vi "Create.vi"(7 "Direction":T1, 8 "error in (no error)":errorcluster, 9 "Custom Config Data":u8[](array[numeric]), 10 "Name":string, 11 "CIFFIFO in":refnum<class "CIF_CIPC_Fifo_DAQ.lvclass">) -> (0 "error out":errorcluster, 3 "CIFFIFO out":refnum<class "CIF_CIPC_Fifo_DAQ.lvclass">)   [LabVIEW 2021, in "CIF_CIPC_Fifo_DAQ.lvclass"]
uses:
  CIF_CIPC_Fifo_DAQ.lvclass
  <vilib>/CIF Foundation/CIF Channels Core/ChannelCommon/typedef/Direction.ctl
  C:/Program Files/National Instruments/LabVIEW 2021/vi.lib/CIF Foundation/CIF Channels Core/CIFChannels/CIFChannels.lvclass
  D:/dev/Packages/CIF_Channels_CIPC/src/CIPC_Channels/CIF_CIPC_Chan/CIF_CIPC_Chn.lvclass
  <vilib>/CIF Foundation/CIF Utilities/Statistics/I64/Stats_I64_CIF_U.lvclass/Stats_I64_CIF_U.ctl
  <vilib>/CIF Foundation/CIF Channels Core/ChannelCommon/typedef/Channel State.ctl
  <vilib>/CIF Foundation/CIF Channels Core/ChannelCommon/typedef/Disconnect Behavior.ctl
  <vilib>/CIF Foundation/CIF Channels Core/CIFChannels/CIFChannels.lvclass/CIFChannels.ctl
  <vilib>/CIF Foundation/CIF Channels Core/ChannelCommon/typedef/Channel Pattern.ctl
  CIF_CIPC_Chan/Typedef/Buffer Configuration Data.ctl
  <vilib>/CIF Foundation/CIF CIPC/TypeDefs/Backpressure References.ctl
  <vilib>/CIF Foundation/CIF CIPC/TypeDefs/Backpressure Names.ctl
  CIF_CIPC_Chan/CIF_CIPC_Chn.lvclass/CIF_CIPC_Chn.ctl
  35849dc3-58aa-4d75-b906-fe3df34869a7.vi
  <vilib>/CIF Foundation/CIF Channels Core/CIFChannels/Accessors/Write Pattern.vi
  CIF_CIPC_Chan/Accessors/Write Buffer Configuration.vi
  CIF_CIPC_Chan/Accessors/Write CIPC Channel.vi
  9be4d617-3037-4515-bcea-2a1e3727d04e.vi
  <vilib>/CIF Foundation/CIF Channels Core/CIFChannels/Accessors/Write Channel State.vi
  <vilib>/CIF Foundation/CIF Channels Core/CIFChannels/Accessors/Write Subscriber Count.vi
  <vilib>/CIF Foundation/CIF Channels Core/CIFChannels/Accessors/Write Channel Benchmark.vi
  <vilib>/CIF Foundation/CIF Channels Core/CIFChannels/Accessors/Write Flatten Benchmark.vi
  35849dc3-58aa-4d75-b906-fe3df34869a7.vi/bd07d5d9-1209-45ad-b636-9e9ab86132fb.vi
  <vilib>/CIF Foundation/CIF CIPC/SubVIs/Check Error.vi
  <vilib>/CIF Foundation/CIF CIPC/SubVIs/Add CIPC Error.vi
  <vilib>/CIF Foundation/CIF CIPC/SubVIs/Get dll Path.vi
  9be4d617-3037-4515-bcea-2a1e3727d04e.vi/49b3dd2d-4579-4089-b72e-3f0875c862f2.vi
  9be4d617-3037-4515-bcea-2a1e3727d04e.vi/1e2c93d0-55b0-4d6c-a9da-21395a664279.vi
  9be4d617-3037-4515-bcea-2a1e3727d04e.vi/7bb13226-97f3-4dcb-9346-06ec631a2876.vi
  9be4d617-3037-4515-bcea-2a1e3727d04e.vi/49b3dd2d-4579-4089-b72e-3f0875c862f2.vi/bd07d5d9-1209-45ad-b636-9e9ab86132fb.vi
  9be4d617-3037-4515-bcea-2a1e3727d04e.vi/1e2c93d0-55b0-4d6c-a9da-21395a664279.vi/49b3dd2d-4579-4089-b72e-3f0875c862f2.vi
  <vilib>/CIF Foundation/CIF CIPC/SubVIs/Notify Of New Write.vi
  <vilib>/CIF Foundation/CIF CIPC/SubVIs/Get Element Write Position.vi
  <vilib>/CIF Foundation/CIF CIPC/SubVIs/Get Element Description Variant.vi
  <vilib>/Utility/error.llb/Trim Whitespace.vi
  <vilib>/string/Create NI GUID.vi
  <vilib>/CIF Foundation/CIF CIPC/SubVIs/Check Error Core.vi
  <vilib>/CIF Foundation/CIF CIPC/SubVIs/Add CIPC Error Core.vi
  <vilib>/CIF Foundation/CIF CIPC/SubVIs/Get Backpressure Name.vi
  <vilib>/CIF Foundation/CIF CIPC/SubVIs/Get Element Info Variant.vi
  <vilib>/CIF Foundation/CIF Utilities/Statistics/I64/Stats_I64_CIF_U.lvclass
  <vilib>/CIF Foundation/CIF Channels Core/CIFChannels/CIFChannels.lvclass
  <vilib>/CIF Foundation/CIF Channels Core/ChannelCommon/ChannelCommon.lvlib
  <vilib>/CIF Foundation/CIF CIPC/CIF_NI_CIPC.lvlib
  CIF_CIPC_Chan/CIF_CIPC_Chn.lvclass
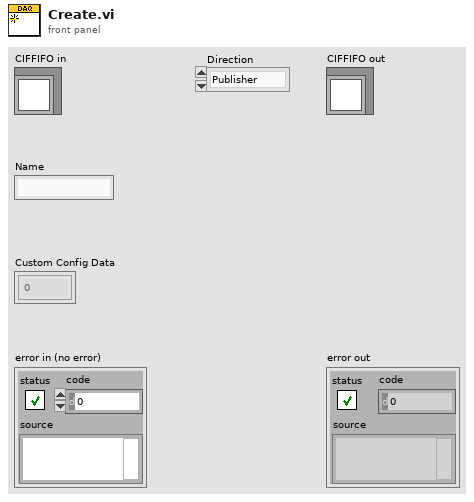
[diagram p1: front panel]
types:
  T1 = typedef "ChannelCommon.lvlib/Direction.ctl" = enum8{"Publisher", "Subscriber"}
  T2 = typedef "ChannelCommon.lvlib/Channel State.ctl" = enum8{"Creating", "Disconnected", "Connecting", "Connected", "Destroyed"}
  T3 = typedef "ChannelCommon.lvlib/Disconnect Behavior.ctl" = enum8{"Default value", "Last value", "Error with default"}
  T4 = typedef "ChannelCommon.lvlib/Channel Pattern.ctl" = enum8{"Unknown", "Tag", "FIFO", "MultiFIFO", "BackpressureFIFO"}
  T5 = typedef "CIF_CIPC_Chn.lvclass/Buffer Configuration Data.ctl" = cluster{"Total Size":u32, "Read Size":u32, "Read Offset":u32, "CIPC BP References":T6, "CIPC Backpressure Names":T7, "Override CIPC Name":string, "Encoder Data":string}
  T6 = typedef "CIF_NI_CIPC.lvlib/Backpressure References.ctl" = cluster{"CIPC Reference":u64, "CIPC BP Reference":u64}
  T7 = typedef "CIF_NI_CIPC.lvlib/Backpressure Names.ctl" = cluster{"CIPC Name":string, "CIPC BP Name":string}
  T8 = typedef "CIF_NI_CIPC.lvlib/Encoder Info.ctl" = cluster{"Name":string, "Version":i32, "Data":string}
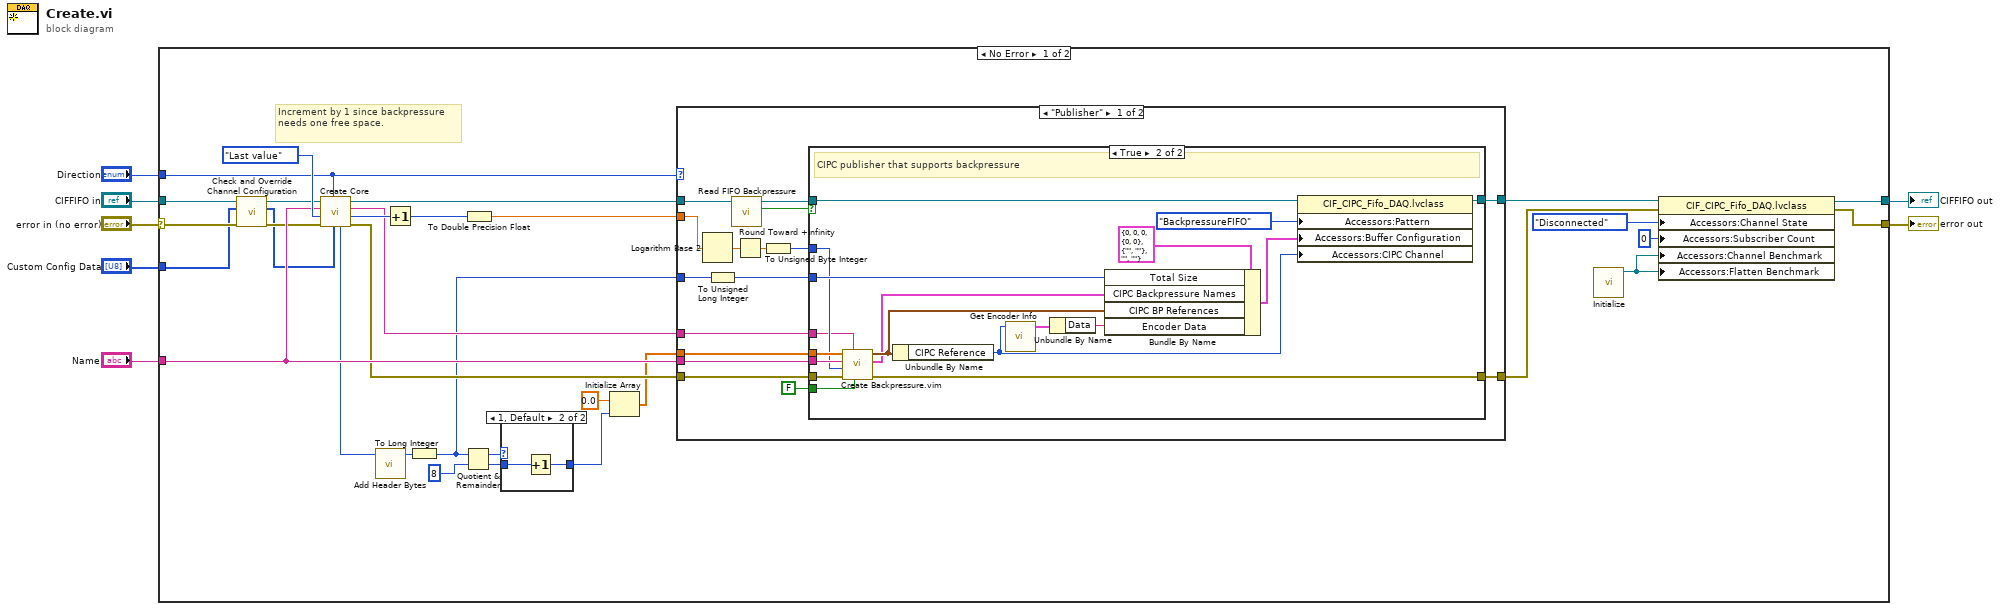
[diagram p0: block diagram]
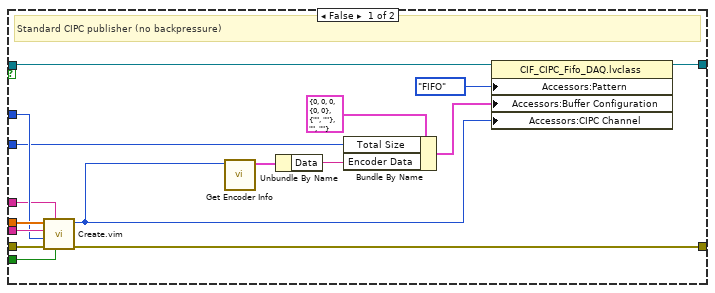
[diagram p3: hidden frame]
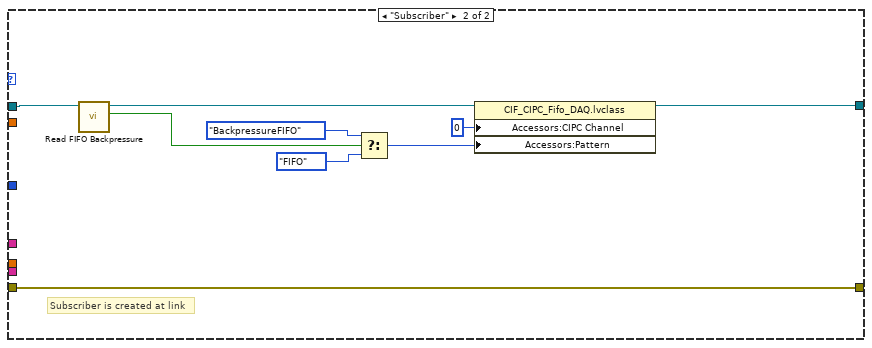
[diagram p4: hidden frame]
diagram:
  n1 = case shown="No Error" "error in (no error)" {
    selector: "error in (no error)" -> [w28 w102]
    tunnel: [w37 w102] -> w6
    tunnel: [w33 w101] -> w1
    tunnel: "CIFFIFO in" -> [w29 w101]
    tunnel: "Name" -> [w36 _]
    tunnel: "Direction" -> [w32 _]
    tunnel: "Custom Config Data" -> [w25 _]
    frame No Error {
      # "Increment by 1 since backpressure needs one free space."
      n2 = call-dynamic "Check and Override Channel Configuration.vi"("error in (no error)"=w28, "Custom Config Data in"=w25, "CIFFIFO in"=w29) -> ("error out"=w26:errorcluster, "Custom Config Data out"=w24:u8[], "CIFFIFO out"=w27:refnum<class "CIF_CIPC_Fifo_DAQ.lvclass">)  [unwired: 6 in]
      n3 = call <vilib>:"Create Core.vi"("Custom Config Data"=w24, "Direction"=w32, "error in (no error)"=w26, "Disconnect Behavior"=Disconnect_Behavior."Last value", "Name"=w36, "CIFChannels in"=w27) -> ("error out"=w35:errorcluster, "Messages"=w19:u64, "Channel Type"=w17:string, "CIFChannels out"=w21:refnum<class "CIF_CIPC_Fifo_DAQ.lvclass">, "Bytes/Msg"=w16:u64)  [unwired: 1 in]
      n4 = call <vilib>:"Add Header Bytes.vi"("Bytes/Msg"=w16) -> ("Bytes/Msg with header"=w20:u64)  [unwired: 3 in]
      n5 = Increment(x=w19) -> (x+1=w18:u64)
      n6 = To Long Integer(number=w20) -> (32bit integer=w15:i32)
      n7 = Quotient & Remainder(x=w15, y=8) -> (x-y*floor(x/y)=w13:i32, floor(x/y)=w12:i32)
      n8 = To Double Precision Float(number=w18) -> (double precision float=w22:dbl)
      n9 = case shown="1, Default" w13 {
        tunnel: w12 -> [w39 w41]
        tunnel: [w39 w40] -> w11
        frame 0 {
        }
        frame 1, Default {
          n10 = Increment(x=w41) -> (x+1=w40:i32)
        }
      }
      n11 = Initialize Array(0.0 ("Numeric"), w11) -> (w23:dbl[])
      n12 = case shown="\"Publisher\"" w32 {
        tunnel: w36 -> [w54 _]
        tunnel: w35 -> [w56 w100]
        tunnel: [w57 w100] -> w34
        tunnel: w22 -> [w51 _]
        tunnel: w23 -> [w53 _]
        tunnel: w21 -> [w48 w94]
        tunnel: w15 -> [w45 _]
        tunnel: [w43 w99] -> w10
        tunnel: w17 -> [w42 _]
        frame "Publisher" {
          n13 = Logarithm Base 2(1:w51) -> (0:w52:dbl)
          n14 = To Unsigned Long Integer(number=w45) -> (unsigned 32bit integer=w44:u32)
          n15 = call <vilib>:"Read FIFO Backpressure.vi"("CIFChannels in"=w48) -> ("Backpressure"=w46:bool, "CIFChannels out"=w47:refnum<class "CIF_CIPC_Fifo_DAQ.lvclass">)  [unwired: 8 in, 1 out]
          n16 = Round Toward +Infinity(x=w52) -> (ceil(x): smallest int >= x=w50:dbl)
          n17 = To Unsigned Byte Integer(number=w50) -> (unsigned 8bit integer=w49:u8)
          n18 = case shown="True" w46 {
            tunnel: [w73 w80] -> w57
            tunnel: w56 -> [w72 w81]
            tunnel: FALSE ("Prepend Array Size") -> [w71 w84]
            tunnel: w54 -> [w70 w83]
            tunnel: w53 -> [w69 w85]
            tunnel: w49 -> [w68 w82]
            tunnel: w47 -> [w67 w91]
            tunnel: w44 -> [w65 w89]
            tunnel: [w61 w86] -> w43
            tunnel: w42 -> [w60 w77]
            frame False {
              # "Standard CIPC publisher (no backpressure)"
              n19 = call "Create.vim"("Prepend Array Size"=w71, "Description"=w60, "error in (no error)"=w72, "Buffer Size N (2^N)"=w68, "Name in"=w70, "Data Type"=w69) -> ("error out"=w73:errorcluster, "CIPC Reference"=w62:u64)  [unwired: 2 in, 2 out]
              n20 = call <vilib>:"Get Encoder Info.vi"("CIPC Reference"=w62) -> ("Encoder Info"=w64:T8)  [unwired: 9 in, 1 out]
              n21 = Unbundle By Name(w64) -> ("Data"=w63:string)
              n22 = Bundle By Name(cluster=T5 {"Total Size"=0, "Read Size"=0, "Read Offset"=0, "CIPC BP References"={"CIPC Reference"=0, "CIPC BP Reference"=0}, "CIPC Backpressure Names"={"CIPC Name"="", "CIPC BP Name"=""}, "Override CIPC Name"="", "Encoder Data"=""} ("Buffer Configuration"), "Total Size"=w65, "Encoder Data"=w63) -> (w59:T5)
              n23 = property class="CIF_CIPC_Fifo_DAQ.lvclass"(reference=w67, "Accessors:Pattern"=Channel_Pattern."FIFO" ("Pattern"), "Accessors:Buffer Configuration"=w59, "Accessors:CIPC Channel"=w62) -> (reference out=w61:refnum<class "CIF_CIPC_Fifo_DAQ.lvclass">)  [unwired: 1 in, 1 out]
            }
            frame True {
              # "CIPC publisher that supports backpressure"
              n24 = call "Create Backpressure.vim"("Prepend Array Size"=w84, "Description"=w77, "error in (no error)"=w81, "Buffer Size N (2^N)"=w82, "Name in"=w83, "Data Type"=w85) -> ("error out"=w80:errorcluster, "CIPC Backpressure Names"=w74:T7, "CIPC BP References"=w78:T6)  [unwired: 2 in, 1 out]
              n25 = Unbundle By Name(w78) -> ("CIPC Reference"=w79:u64)
              n26 = call <vilib>:"Get Encoder Info.vi"("CIPC Reference"=w79) -> ("Encoder Info"=w88:T8)  [unwired: 9 in, 1 out]
              n27 = Unbundle By Name(w88) -> ("Data"=w87:string)
              n28 = Bundle By Name(cluster=T5 {"Total Size"=0, "Read Size"=0, "Read Offset"=0, "CIPC BP References"={"CIPC Reference"=0, "CIPC BP Reference"=0}, "CIPC Backpressure Names"={"CIPC Name"="", "CIPC BP Name"=""}, "Override CIPC Name"="", "Encoder Data"=""} ("Buffer Configuration"), "Total Size"=w89, "CIPC Backpressure Names"=w74, "CIPC BP References"=w78, "Encoder Data"=w87) -> (w76:T5)
              n29 = property class="CIF_CIPC_Fifo_DAQ.lvclass"(reference=w91, "Accessors:Pattern"=Channel_Pattern."BackpressureFIFO" ("Pattern"), "Accessors:Buffer Configuration"=w76, "Accessors:CIPC Channel"=w79) -> (reference out=w86:refnum<class "CIF_CIPC_Fifo_DAQ.lvclass">)  [unwired: 1 in, 1 out]
            }
          }
        }
        frame "Subscriber" {
          # "Subscriber is created at link"
          n30 = call <vilib>:"Read FIFO Backpressure.vi"("CIFChannels in"=w94) -> ("Backpressure"=w95:bool, "CIFChannels out"=w93:refnum<class "CIF_CIPC_Fifo_DAQ.lvclass">)  [unwired: 8 in, 1 out]
          n31 = Select(t=Channel_Pattern."BackpressureFIFO" ("Pattern"), s=w95, f=Channel_Pattern."FIFO" ("Pattern")) -> (s? t:f=w92:T4)
          n32 = property class="CIF_CIPC_Fifo_DAQ.lvclass"(reference=w93, "Accessors:CIPC Channel"=u64 0 ("CIPC Channel"), "Accessors:Pattern"=w92) -> (reference out=w99:refnum<class "CIF_CIPC_Fifo_DAQ.lvclass">)  [unwired: 1 in, 1 out]
        }
      }
      n33 = call <vilib>:"Initialize.vi"() -> ("Stats_I64_CIF_U out"=w30:refnum<class "Stats_I64_CIF_U.lvclass">)  [unwired: 10 in, 1 out]
      n34 = property class="CIF_CIPC_Fifo_DAQ.lvclass"(reference=w10, error in=w34, "Accessors:Channel State"=Channel_State."Disconnected" ("Channel State"), "Accessors:Subscriber Count"=u32 0 ("Subscriber Count"), "Accessors:Channel Benchmark"=w30, "Accessors:Flatten Benchmark"=w30) -> (reference out=w33:refnum<class "CIF_CIPC_Fifo_DAQ.lvclass">, error out=w37:errorcluster)
    }
    frame Error {
    }
  }
  "error out" <- w6
  "CIFFIFO out" <- w1
